vi "Engine Daemon Async.vi"(10 "Daemon Notifier":refnum<notifier>, 11 "TSEngine in":refnum<class "Engine.lvclass">) -> ()   [LabVIEW 2020, in "TSS.lvlib" / "Engine.lvclass"]
uses:
  Engine.lvclass
  Engine.lvclass/Engine.ctl
  Typedefs/Session Handle.ctl
  Session Notification.ctl
  d09647a5-81ab-4110-adb4-612663b1efb2.vi
  VariableContainer/VariableContainer.lvclass
  SequenceFile/SequenceFile.lvclass
  Execution/Execution.lvclass
panel:
  out "error out":errorcluster
  out "Log":string
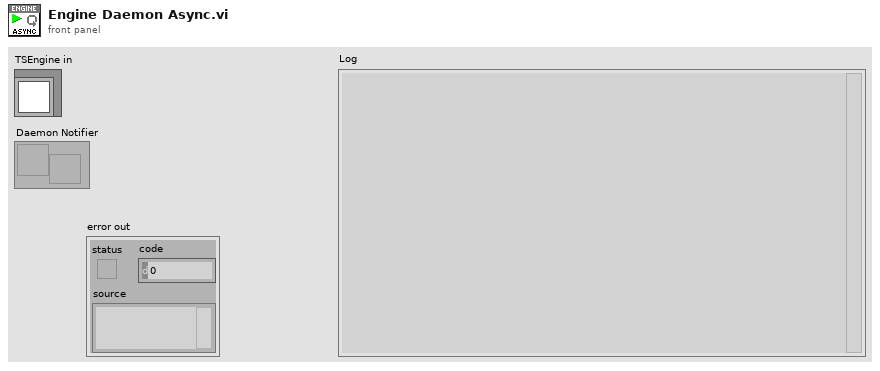
[diagram p1: front panel]
types:
  T1 = enum32{"Invalid", "Standard", "Closed", "Hidden", "Minimized", "Maximized"}
  T2 = enum32{"invalid app kind", "Development System", "Run Time System", "Student Edition", "Embedded LabVIEW", "Evaluation", "Custom"}
  T3 = typedef "TSS.lvlib/Engine.lvclass/Events.ctl" = cluster{"Stop Deamon":refnum<user-event>, "Create Variable Container":refnum<user-event>, "Create Report":refnum<user-event>, "Open Sequence File":refnum<user-event>, "Prepare Execution":refnum<user-event>}
  T4 = typedef "TSS.lvlib/Engine.lvclass/Session Notification.ctl" = cluster{"Session":refnum<data-value>, "Error":errorcluster}
  T5 = typedef "TSS.lvlib/Engine.lvclass/Session Handle.ctl" = refnum<data-value>
  T6 = typedef "TSS.lvlib/Execution.lvclass/Execution Options.ctl" = cluster{"Use Default Model":bool}
  T7 = typedef "TSS.lvlib/Execution.lvclass/Session Handle.ctl" = refnum<data-value>
  T8 = typedef "TSS.lvlib/Report.lvclass/Session Handle.ctl" = refnum<data-value>
  T9 = typedef "TSS.lvlib/File Load Options.ctl" = cluster{"Use Search Dirs? (T)":bool, "Conflict as Error? (T)":bool, "Check Station Model? (F)":bool, "Preload Modules? (T)":bool, "Skip Load Callback? (F)":bool, "Reload if Loaded? (F)":bool}
  T10 = typedef "TSS.lvlib/SequenceFile.lvclass/Session Handle.ctl" = refnum<data-value>
  T11 = typedef "TSS.lvlib/Engine.lvclass/Variable Container Type.ctl" = enum16{"StationGlobals", "TemporaryGlobals", "NewPropertyObject"}
  T12 = typedef "TSS.lvlib/VariableContainer.lvclass/Session Handle.ctl" = refnum<data-value>
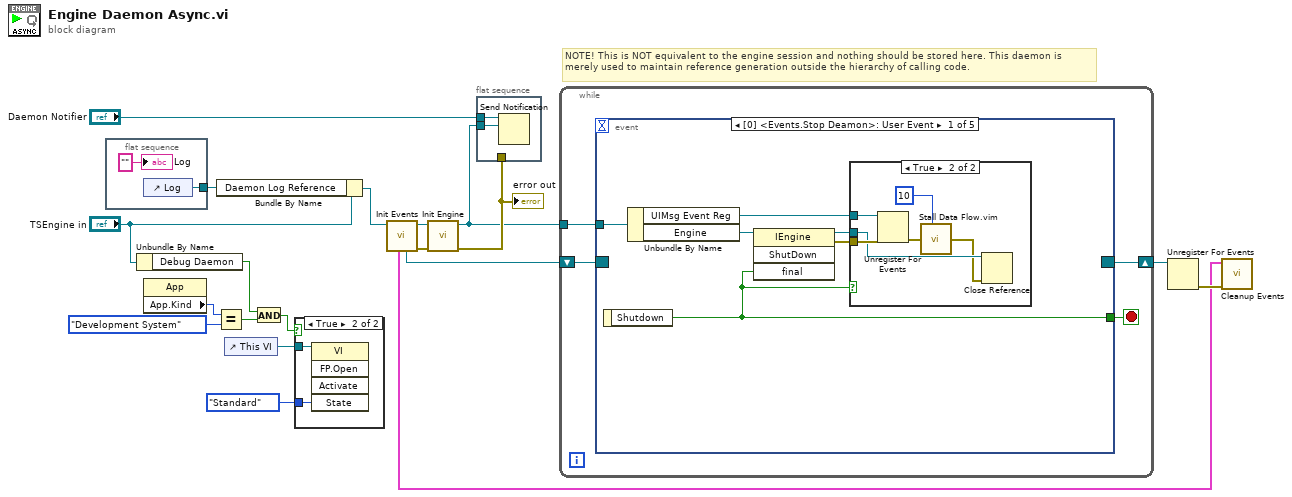
[diagram p0: block diagram]
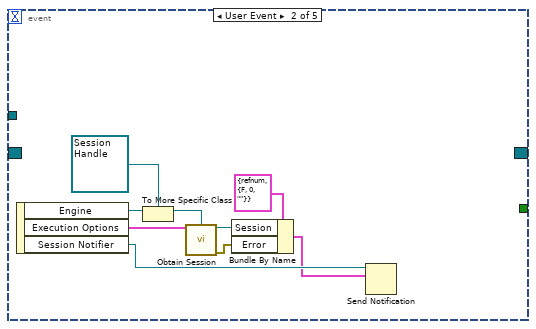
[diagram p4: hidden frame]
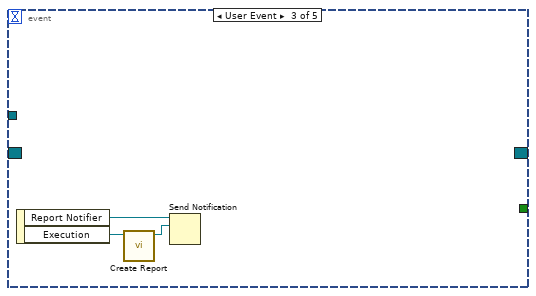
[diagram p5: hidden frame]
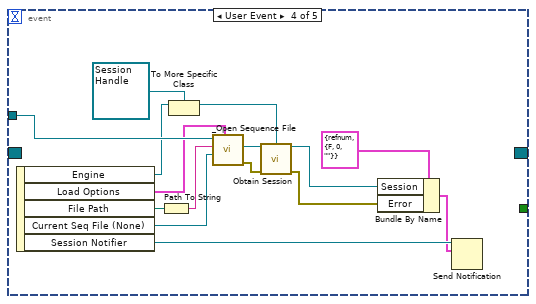
[diagram p6: hidden frame]
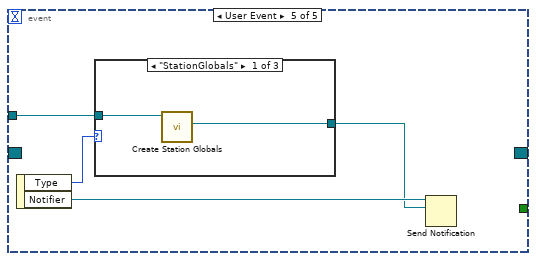
[diagram p7: hidden frame]
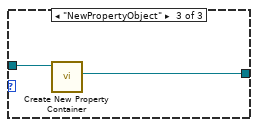
[diagram p9: hidden frame]
diagram:
  # "NOTE! This is NOT equivalent to the engine session and nothing should be stored here. This daemon is merely used to maintain reference generation outside the hierarchy of calling code."
  n1 = flat-sequence {
    tunnel: [w21] -> w9
    frame #0 {
      n2 = control-ref of="Log"() -> (w21:refnum<vi>)
      "Log" <- "" ("Log")
    }
  }
  n3 = Unbundle By Name("TSEngine in") -> ("Debug Daemon"=w4:bool)
  n4 = property class="App"() -> ("App.Kind"=w8:T2)  [unwired: 2 in, 2 out]
  n5 = Equal?(x=w8, y=T2."Development System") -> (x = y?=w5:bool)
  n6 = Bundle By Name(cluster="TSEngine in", "Daemon Log Reference"=w9) -> (w10:refnum<class "Engine.lvclass">)
  n7 = control-ref of="This VI"() -> (w3:refnum<vi>)
  n8 = And(x=w4, y=w5) -> (x .and. y?=w1:bool)
  n9 = case shown="True" w1 {
    tunnel: w3 -> [_ w23]
    tunnel: T1."Standard" ("State") -> [_ w22]
    frame False {
    }
    frame True {
      n10 = invoke class="VI" method="FP.Open"(reference=w23, "State"=w22) -> ()  [unwired: 3 in, 5 out]
    }
  }
  n11 = call "Init Events.vi"("TSEngine in"=w10) -> ("error out"=w14:errorcluster, "TSEngine out"=w15:refnum<class "Engine.lvclass">, "Event Reg"=w13:refnum<event-registration>, "Events"=w11:T3)  [unwired: 7 in]
  n12 = call "Init Engine.vi"("error in (no error)"=w14, "TSEngine in"=w15) -> ("error out"=w19:errorcluster, "TSEngine out"=w16:refnum<class "Engine.lvclass">)  [unwired: 8 in]
  "error out" <- w19
  n13 = flat-sequence {
    tunnel: "Daemon Notifier" -> [w25]
    tunnel: w16 -> [w24]
    tunnel: w19 -> [_]
    frame #0 {
      n14 = Send Notification(notification=w24, notifier=w25) -> ()  [unwired: 1 in, 2 out]
    }
  }
  n15 = while {
    shift-right: [w28] -> w17
    shift-left: w13 -> [w29]
    tunnel: w16 -> [w26]
    stop <- w27 stop-if-true
    n16 = event shown="[0] <Events.Stop Deamon>: User Event" {
      selector: w29 -> [_ _ _ _ _]
      dyn-events: [_ _ _ _ _] -> w28
      timeout: _ -> [_ _ _ _ _]
      tunnel: [w30 _ _ _ _] -> w27
      tunnel: w26 -> [w35 _ _ w68 w71]
      event User Event {
        n17 = event-data() -> ("Shutdown"=w30:bool)  [unwired: 1 in]
        n18 = Unbundle By Name(w35) -> ("UIMsg Event Reg"=w31:refnum<k27>, "Engine"=w34:refnum<k7>)
        n19 = invoke class="IEngine" method="ShutDown"(reference=w34, "final"=w30) -> (reference out=w33:refnum<k7>, error out=w32:errorcluster)  [unwired: 2 in, 2 out]
        n20 = case shown="True" w30 {
          tunnel: w33 -> [_ w38]
          tunnel: w32 -> [_ w39]
          tunnel: w31 -> [_ w40]
          frame False {
          }
          frame True {
            n21 = Unregister For Events(event registration refnum=w40, error in=w39) -> (error out=w41:errorcluster)
            n22 = call "Stall Data Flow.vim"("value in"=w41, "milliseconds to wait"=u32 10) -> ("value out"=w37:errorcluster)  [unwired: 1 out]
            n23 = Close Reference(reference=w38, error in (no error)=w37) -> ()  [unwired: 1 out]
          }
        }
      }
      event User Event {
        n24 = event-data() -> ("Engine"=w49:refnum<data-value>, "Execution Options"=w50:T6, "Session Notifier"=w46:refnum<notifier>)  [unwired: 1 in]
        n25 = To More Specific Class(target class=T5 refnum ("Engine"), reference=w49) -> (specific class reference=w48:T5)  [unwired: 1 in, 1 out]
        n26 = call "Obtain Session.vi"("Options"=w50, "Engine"=w48) -> ("Session Handle"=w43:T7, "error out"=w42:errorcluster)  [unwired: 12 in]
        n27 = Bundle By Name(cluster=T4 {"Session"=refnum, "Error"={"status"=FALSE, "code"=0, "source"=""}} ("notification"), "Session"=w43, "Error"=w42) -> (w44:T4)
        n28 = Send Notification(notification=w44, notifier=w46) -> ()  [unwired: 1 in, 2 out]
      }
      event User Event {
        n29 = event-data() -> ("Report Notifier"=w52:refnum<notifier>, "Execution"=w53:T7)  [unwired: 1 in]
        n30 = call "Create Report.vi"("Execution"=w53) -> ("Report"=w51:T8)  [unwired: 9 in, 1 out]
        n31 = Send Notification(notification=w51, notifier=w52) -> ()  [unwired: 1 in, 2 out]
      }
      event User Event {
        n32 = event-data() -> ("Engine"=w60:refnum<data-value>, "Load Options"=w67:T9, "File Path"=w66:path, "Current Seq File (None)"=w64:T10, "Session Notifier"=w63:refnum<notifier>)  [unwired: 1 in]
        n33 = Path To String(path=w66) -> (string=w65:string)
        n34 = To More Specific Class(target class=T5 refnum ("Engine"), reference=w60) -> (specific class reference=w57:T5)  [unwired: 1 in, 1 out]
        n35 = call "_Open Sequence File.vi"("Load Options"=w67, "Current Seq File (None)"=w64, "File Path"=w65, "Engine in"=w68) -> ("error out"=w56:errorcluster, "SeqFile Ref"=w58:refnum<k7>)  [unwired: 5 in, 1 out]
        n36 = call "Obtain Session.vi"("SequenceFile"=w58, "Engine"=w57, "error in (no error)"=w56) -> ("Session Handle"=w54:T10, "error out"=w55:errorcluster)  [unwired: 11 in]
        n37 = Bundle By Name(cluster=T4 {"Session"=refnum, "Error"={"status"=FALSE, "code"=0, "source"=""}} ("notification"), "Session"=w54, "Error"=w55) -> (w61:T4)
        n38 = Send Notification(notification=w61, notifier=w63) -> ()  [unwired: 1 in, 2 out]
      }
      event User Event {
        n39 = event-data() -> ("Type"=w72:T11, "Notifier"=w70:refnum<notifier>)  [unwired: 1 in]
        n40 = case shown="\"StationGlobals\"" w72 {
          tunnel: w71 -> [w74 _ w76]
          tunnel: [w73 _ w75] -> w69
          frame "StationGlobals" {
            n41 = call "Create Station Globals.vi"("TSEngine in"=w74) -> ("StationGlobals"=w73:T12)  [unwired: 8 in, 2 out]
          }
          frame "TemporaryGlobals" {
            # "#TODO\nTemporary Globals"
          }
          frame "NewPropertyObject" {
            n42 = call "Create New Property Container.vi"("Engine in"=w76) -> ("PropertyObject"=w75:T12)  [unwired: 8 in, 2 out]
          }
        }
        n43 = Send Notification(notification=w69, notifier=w70) -> ()  [unwired: 1 in, 2 out]
      }
    }
  }
  n44 = Unregister For Events(event registration refnum=w17) -> (error out=w12:errorcluster)  [unwired: 1 in]
  n45 = call "Cleanup Events.vi"("error in (no error)"=w12, "Events"=w11) -> ()  [unwired: 10 in]
